vi "波形编辑.vi"(11 "db file":path=path "D:/Data/波形.sqlite3") -> (3 "波形图":waveform(dbl)(graph))   [LabVIEW 2020, in "功能选择.xctl"]
uses:
  <vilib>/drjdpowell/SQLite Library/SQL Statement/SQL Statement.lvclass/SQL Statement.ctl
  <vilib>/drjdpowell/SQLite Library/SQL Connection/Open (path).vi
  <vilib>/drjdpowell/SQLite Library/SQL Statement/Bind Text.vi
  <vilib>/drjdpowell/SQLite Library/SQL Statement/First Step.vi
  <vilib>/drjdpowell/SQLite Library/SQL Statement/Column DBL.vi
  <vilib>/drjdpowell/SQLite Library/SQL Statement/Finalize (Property).vi
  <vilib>/drjdpowell/SQLite Library/SQL Connection/Open (string).vi
  <vilib>/drjdpowell/SQLite Library/SQL Statement/Step.vi
  <vilib>/drjdpowell/SQLite Library/SQL Statement/Column Type.vi
  <vilib>/drjdpowell/SQLite Library/SQL Statement/Finalize.vi
  <vilib>/AdvancedString/Path To Command Line String.vi
  <vilib>/drjdpowell/SQLite Library/SQL Connection/Execute SQL (No results).vi
  <vilib>/Utility/file.llb/Write Delimited Spreadsheet (string).vi
  <vilib>/Utility/file.llb/Read Delimited Spreadsheet (string).vi
  <vilib>/drjdpowell/SQLite Library/SQL Statement/Error Message.vi
  <vilib>/drjdpowell/SQLite Library/SQL Statement/Column String.vi
  <vilib>/drjdpowell/SQLite Library/SQL Connection/Execute SQL (1D String).vi
  <vilib>/drjdpowell/SQLite Library/SQL Connection/Connection.lvclass
  <vilib>/drjdpowell/SQLite Library/SQL Statement/SQL Statement.lvclass
  <vilib>/drjdpowell/SQLite Library/SQLite.lvlib
panel:
  in  "limit I":dbl=0.01 min=1e-08 max=3.0 format="%#_6pA"
  in  "搜索":string
  out "保存列表":i32(listbox)
  in  "采样点（秒/个）":dbl=0.001 min=6.5e-05 max=1.0 step=1e-06 format="%#_6ps"
  in  "波形描述":string[][](table)=[["--------", "--end--", "--------", "--------"]]
  # "类型：\nL=线性  log=对数\nP=脉冲  S=阶跃"
  # "类型为对数时备注为渐近线线\n         脉冲时为占空比0-100\n         阶跃信号为突变位置0-100"
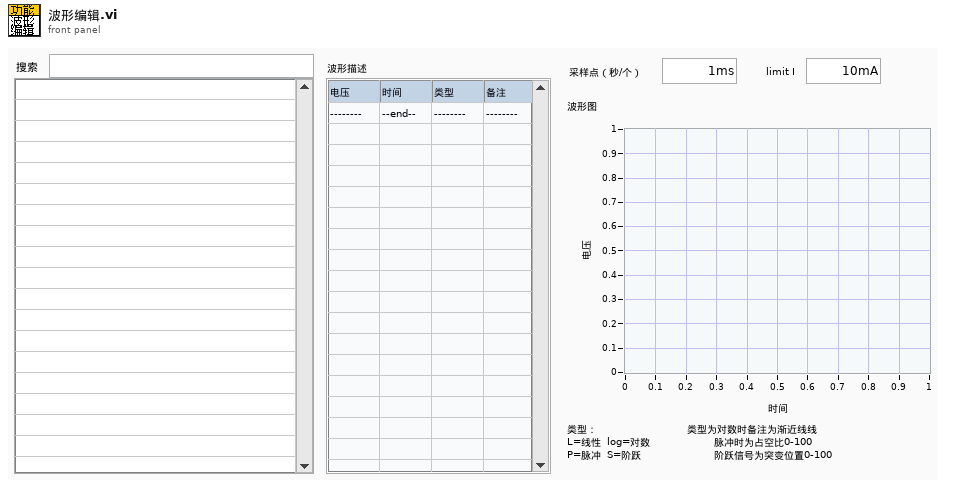
[diagram p1: front panel]
types:
  T1 = cluster{string, "采样点（秒/个）":dbl, "JSON string":string}
  T2 = typedef "LVPoint32TypeDef.ctl" = cluster{"Horizontal":i32, "Vertical":i32}
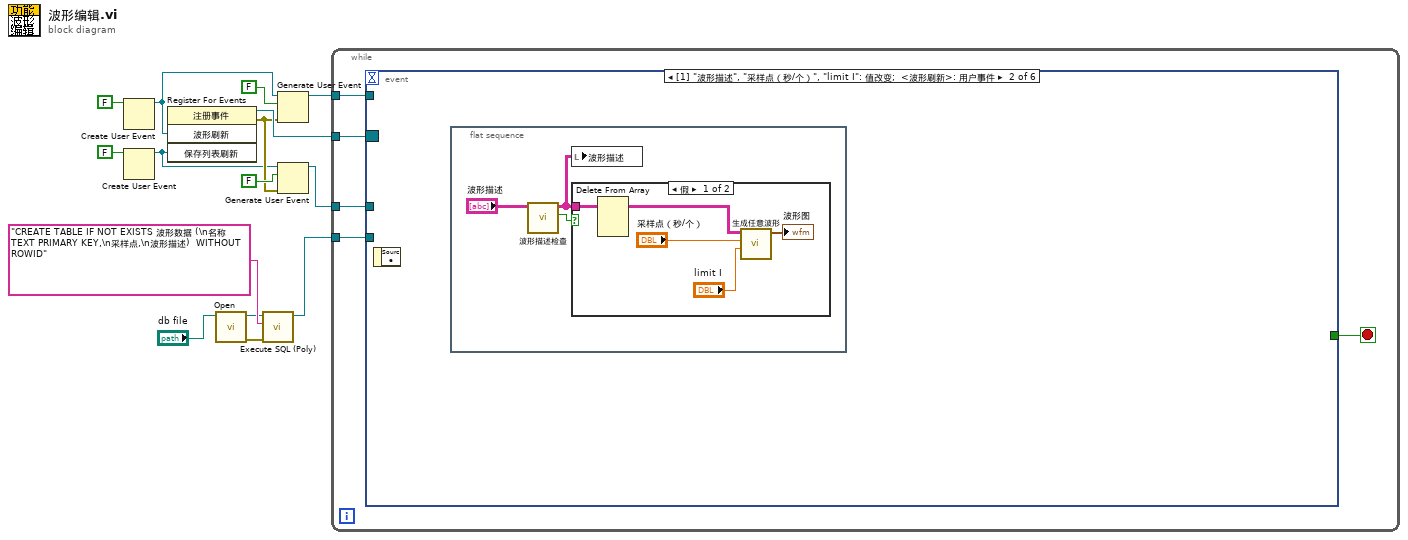
[diagram p0: block diagram]
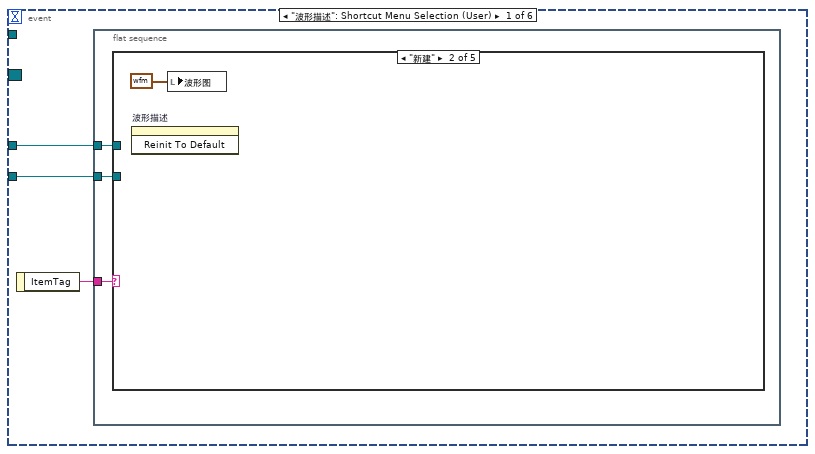
[diagram p2: hidden frame]
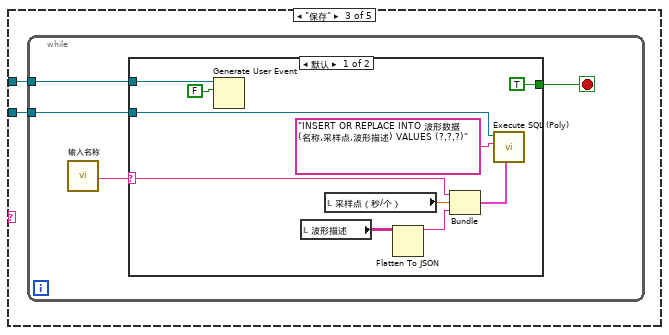
[diagram p4: hidden frame]
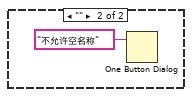
[diagram p5: hidden frame]
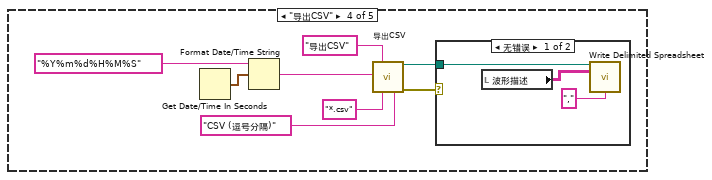
[diagram p6: hidden frame]
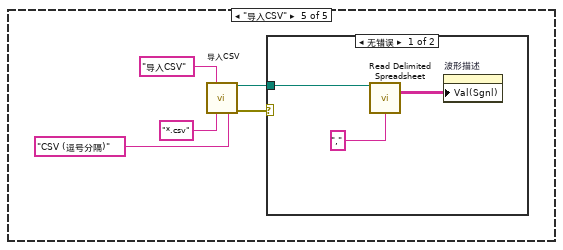
[diagram p8: hidden frame]
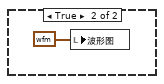
[diagram p10: hidden frame]
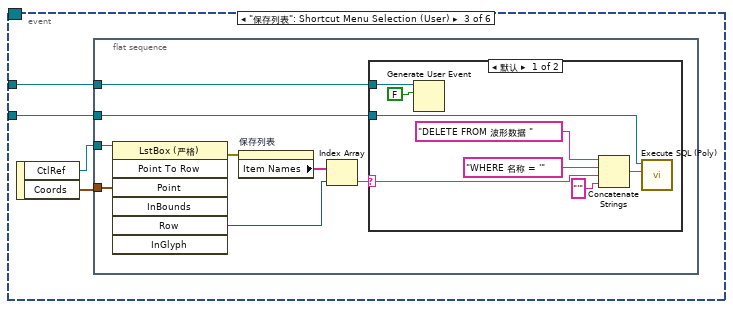
[diagram p11: hidden frame]
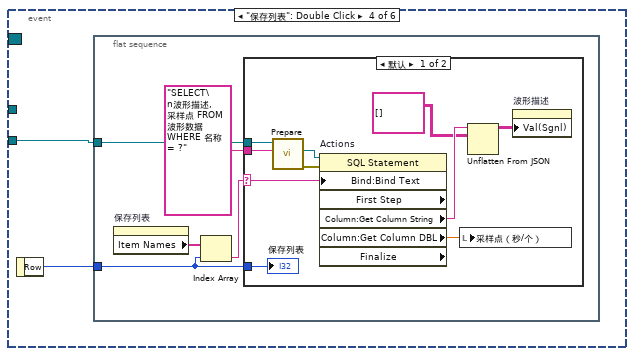
[diagram p13: hidden frame]
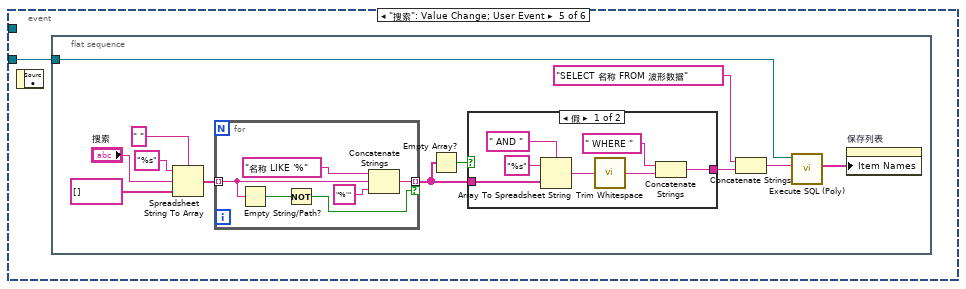
[diagram p15: hidden frame]
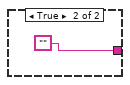
[diagram p16: hidden frame]
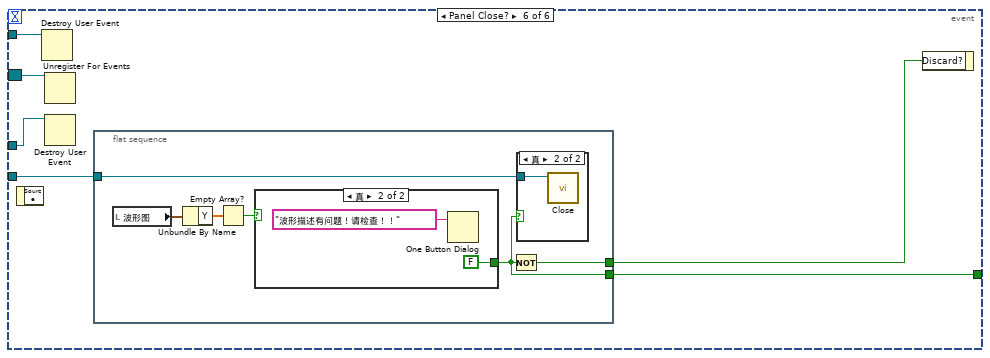
[diagram p17: hidden frame]
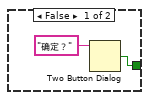
[diagram p19: hidden frame]
diagram:
  n1 = Create User Event(user event datatype=FALSE ("波形刷新")) -> (user event=w5:refnum<user-event>)  [unwired: 1 in, 1 out]
  n2 = Create User Event(user event datatype=FALSE ("保存列表刷新")) -> (user event=w3:refnum<user-event>)  [unwired: 1 in, 1 out]
  n3 = register-events(w5, w3) -> (reference out=w9:refnum<event-registration>, error out=w4:errorcluster)  [unwired: 2 in]
  n4 = call-poly <vilib>:"Open.vi"("db file"="db file") -> ("error out"=w11:errorcluster, "SQLite Connection"=w13:refnum<class "Connection.lvclass">)  [unwired: 9 in]
  n5 = call-poly <vilib>:"Execute SQL (Poly).vi"("error in (no error)"=w11, "SQL"="CREATE TABLE IF NOT EXISTS 波形数据 (\n名称 TEXT PRIMARY KEY,\n采样点,\n波形描述)  WITHOUT ROWID", "SQLite Connection in"=w13) -> ("SQLite Connection"=w12:refnum<class "Connection.lvclass">)  [unwired: 7 in, 1 out]
  n6 = Generate User Event(user event=w5, event data cluster=FALSE ("事件数据"), error in=w4) -> (user event out=w1:refnum<user-event>)  [unwired: 1 in, 1 out]
  n7 = Generate User Event(user event=w3, event data cluster=FALSE ("事件数据"), error in=w4) -> (user event out=w2:refnum<user-event>)  [unwired: 1 in, 1 out]
  n8 = while {
    tunnel: w12 -> [w19]
    tunnel: w9 -> [w18]
    tunnel: w2 -> [w17]
    tunnel: w1 -> [w16]
    stop <- w20 stop-if-true
    n9 = event shown="[1] \"波形描述\", \"采样点（秒/个）\", \"limit I\": 值改变;  <波形刷新>: 用户事件" {
      selector: w18 -> [_ _ _ _ _ w139]
      dyn-events: _ -> [_ _ _ _ _ _]
      timeout: _ -> [_ _ _ _ _ _]
      tunnel: [_ _ _ _ _ w141] -> w20
      tunnel: w19 -> [w22 _ w74 w93 w110 w142]
      tunnel: w17 -> [w21 _ w73 _ _ w138]
      tunnel: w16 -> [_ _ _ _ _ w137]
      event "波形描述": Shortcut Menu Selection (User) {
        n10 = event-data() -> ("ItemTag"=w23:string)  [unwired: 1 in]
        n11 = flat-sequence {
          tunnel: w23 -> [w26]
          tunnel: w22 -> [w25]
          tunnel: w21 -> [w24]
          frame #0 {
            n12 = case shown="\"新建\"" w26 {
              tunnel: w25 -> [_ _ w29 _ _]
              tunnel: w24 -> [_ _ w28 _ _]
              frame Default {
              }
              frame "新建" {
                n13 = invoke on="波形描述" class="Tbl (严格)" method="Reinit To Default"() -> ()  [unwired: 3 in, 3 out]
                n14 = local write "波形图"(waveform(dbl) {"t0"=timestamp(0 s since 1904-01-01), "dt"=1.0, "Y"=[]} ("波形图")) -> ()
              }
              frame "保存" {
                n15 = while {
                  tunnel: w29 -> [w33]
                  tunnel: w28 -> [w30]
                  stop <- w31 stop-if-true
                  n16 = call "输入名称"() -> ("名称"=w32:string)  [unwired: 17 in, 2 out]
                  n17 = case shown="默认" w32 {
                    selector: w32 -> [w36 _]
                    tunnel: w33 -> [w38 _]
                    tunnel: [TRUE _] -> w31
                    tunnel: w30 -> [w35 _]
                    frame Default {
                      n18 = Generate User Event(user event=w35, event data cluster=FALSE ("事件数据")) -> ()  [unwired: 2 in, 2 out]
                      n19 = local read "波形描述"() -> (w40:string[][])
                      n20 = local read "采样点（秒/个）"() -> (w42:dbl)
                      n21 = Flatten To JSON(anything=w40) -> (JSON string=w41:string)  [unwired: 2 in, 1 out]
                      n22 = Bundle(w36, "采样点（秒/个）"=w42, "JSON string"=w41) -> (w43:T1)  [unwired: 1 in]
                      n23 = call-poly <vilib>:"Execute SQL (Poly).vi"("Parameter(s)"=w43, "SQL"="INSERT OR REPLACE INTO 波形数据 (名称,采样点,波形描述) VALUES (?,?,?)", "SQLite Connection in"=w38) -> ()  [unwired: 7 in, 2 out]
                    }
                    frame "" {
                      n24 = One Button Dialog(message="不允许空名称" ("消息")) -> ()  [unwired: 1 in, 1 out]
                    }
                  }
                }
              }
              frame "导出CSV" {
                n25 = Get Date/Time In Seconds() -> (seconds since 1Jan1904=w49:timestamp)
                n26 = Format Date/Time String(time format string (%c)="%Y%m%d%H%M%S" ("时间格式字符串(%c)"), seconds (now)=w49) -> (date/time string=w48:string)  [unwired: 1 in]
                n27 = call "导出CSV"("prompt"="导出CSV", "default name"=w48, "pattern (all files)"="*.csv" ("pattern label"), "pattern label"="CSV (逗号分隔)" ("pattern (all files)")) -> ("selected path"=w52:path, "error out"=w46:errorcluster)  [unwired: 8 in, 2 out]
                n28 = case shown="无错误" w46 {
                  tunnel: w52 -> [w55 _]
                  frame No Error {
                    n29 = local read "波形描述"() -> (w54:string[][])
                    n30 = call-poly <vilib>:"Write Delimited Spreadsheet.vi"("file path (dialog if empty)"=w55, "2D data"=w54, "delimiter (\\t)"="," ("delimiter (\\t)")) -> ()  [unwired: 11 in, 2 out]
                  }
                  frame Error {
                  }
                }
              }
              frame "导入CSV" {
                n31 = call "导入CSV"("prompt"="导入CSV", "pattern (all files)"="*.csv" ("pattern label"), "pattern label"="CSV (逗号分隔)" ("pattern (all files)")) -> ("selected path"=w60:path, "error out"=w59:errorcluster)  [unwired: 9 in, 2 out]
                n32 = case shown="无错误" w59 {
                  tunnel: w60 -> [w63 _]
                  frame No Error {
                    n33 = call-poly <vilib>:"Read Delimited Spreadsheet.vi"("file path (dialog if empty)"=w63, "delimiter (\\t)"="," ("delimiter (\\t)")) -> ("all rows"=w61:string[][])  [unwired: 8 in, 5 out]
                    n34 = property on="波形描述" class="Tbl (严格)"("Val(Sgnl)"=w61) -> ()  [unwired: 2 in, 2 out]
                  }
                  frame Error {
                  }
                }
              }
            }
          }
        }
      }
      event "波形描述", "采样点（秒/个）", "limit I": Value Change; User Event {
        n35 = event-data() -> ()  [unwired: 1 in, 1 out]
        n36 = flat-sequence {
          frame #0 {
            n37 = call "波形描述检查.vi"("波形描述"="波形描述") -> ("正确"=w66:bool, "波形描述输出"=w64:string[][])  [unwired: 9 in]
            n38 = local write "波形描述"(w64) -> ()
            n39 = case shown="假" w66 {
              tunnel: w64 -> [w67 _]
              frame False {
                n40 = Delete From Array(array=w67) -> (array with subset deleted=w68:string[][])  [unwired: 3 in, 1 out]
                n41 = call "生成任意波形.vi"("限流"="limit I", "采样点"="采样点（秒/个）", "波形描述"=w68) -> ("波形图"=→"波形图":waveform(dbl))  [unwired: 8 in]
              }
              frame True {
                n42 = local write "波形图"(waveform(dbl) {"t0"=timestamp(0 s since 1904-01-01), "dt"=1.0, "Y"=[]} ("Waveform")) -> ()
              }
            }
          }
        }
      }
      event "保存列表": Shortcut Menu Selection (User) {
        n43 = event-data() -> ("CtlRef"=w76:refnum<vi>, "Coords"=w75:T2)  [unwired: 1 in]
        n44 = flat-sequence {
          tunnel: w76 -> [w84]
          tunnel: w75 -> [w83]
          tunnel: w74 -> [w79]
          tunnel: w73 -> [w77]
          frame #0 {
            n45 = invoke class="LstBox (严格)" method="Point To Row"(reference=w84, "Point"=w83) -> (error out=w78:errorcluster, "Row"=w81:i32)  [unwired: 5 in, 5 out]
            n46 = property on="保存列表" class="LstBox (严格)"(error in=w78) -> ("Item Names"=w82:string[])  [unwired: 1 in, 2 out]
            n47 = Index Array(array=w82, index=w81) -> (element=w80:string)
            n48 = case shown="默认" w80 {
              selector: w80 -> [w90 _]
              tunnel: w79 -> [w89 _]
              tunnel: w77 -> [w86 _]
              frame Default {
                n49 = Generate User Event(user event=w86, event data cluster=FALSE ("事件数据")) -> ()  [unwired: 2 in, 2 out]
                n50 = Concatenate Strings("DELETE FROM 波形数据 " ("字符串"), "WHERE 名称 = '" ("condition"), w90, "'" ("字符串")) -> (w87:string)
                n51 = call-poly <vilib>:"Execute SQL (Poly).vi"("SQL"=w87, "SQLite Connection in"=w89) -> ()  [unwired: 8 in, 2 out]
              }
              frame "" {
              }
            }
          }
        }
      }
      event "保存列表": Double Click {
        n52 = event-data() -> ("Row"=w94:i32)  [unwired: 1 in]
        n53 = flat-sequence {
          tunnel: w94 -> [w99]
          tunnel: w93 -> [w96]
          frame #0 {
            n54 = property on="保存列表" class="LstBox (严格)"() -> ("Item Names"=w98:string[])  [unwired: 2 in, 2 out]
            n55 = Index Array(array=w98, index=w99) -> (element=w97:string)
            n56 = case shown="默认" w97 {
              selector: w97 -> [w104 _]
              tunnel: w99 -> [w109 _]
              tunnel: w96 -> [w105 _]
              tunnel: "SELECT\n波形描述, 采样点 FROM 波形数据 WHERE 名称 = ?" ("SELECT  statement") -> [w102 _]
              frame Default {
                n57 = call <vilib>:"Prepare.vi"("SQL"=w102, "SQLite Connection in"=w105) -> ("error out"=w106:errorcluster, "SQL Statement"=w107:refnum<class "SQL Statement.lvclass">)  [unwired: 5 in, 3 out]
                n58 = property on="Actions" class="SQL Statement" props=["Bind:Bind Text", "First Step", "Column:Get Column String", "Column:Get Column DBL", "Finalize"](reference=w107, error in=w106, "Bind:Bind Text"=w104) -> ("Column:Get Column String"=w103:string, "Column:Get Column DBL"=w101:dbl)  [unwired: 4 out]
                n59 = local write "采样点（秒/个）"(w101) -> ()
                n60 = Unflatten From JSON(JSON string=w103, type and defaults=string[][] []) -> (value=w108:string[][])  [unwired: 5 in, 1 out]
                n61 = property on="波形描述" class="Tbl (严格)"("Val(Sgnl)"=w108) -> ()  [unwired: 2 in, 2 out]
                "保存列表" <- w109
              }
              frame "" {
              }
            }
          }
        }
      }
      event "搜索": Value Change; User Event {
        n62 = event-data() -> ()  [unwired: 1 in, 1 out]
        n63 = flat-sequence {
          tunnel: w110 -> [w111]
          frame #0 {
            n64 = Spreadsheet String To Array(delimiter (Tab)=" " ("分隔符(Tab)"), format string="%s" ("格式字符串"), spreadsheet string="搜索", array type (2D Dbl)=string[] []) -> (array=w118:string[])
            n65 = for {
              tunnel: w118 -> [w133] mode=indexing
              tunnel: [w134] -> w117 mode=indexing if=w131
              n66 = Empty String/Path?(string/path=w133) -> (empty?=w132:bool)
              n67 = Not(x=w132) -> (.not. x?=w131:bool)
              n68 = Concatenate Strings("名称 LIKE '%" ("字符串"), w133, "%'" ("condition")) -> (w134:string)
            }
            n69 = Empty Array?(array=w117) -> (empty?=w116:bool)
            n70 = case shown="假" w116 {
              tunnel: [w125 ""] -> w112
              tunnel: w117 -> [w123 _]
              frame False {
                n71 = Array To Spreadsheet String(delimiter (Tab)=" AND " ("分隔符(Tab)"), array=w123, 3:"%s" ("格式字符串")) -> (spreadsheet string=w127:string)
                n72 = call <vilib>:"Trim Whitespace.vi"("string"=w127) -> ("trimmed string"=w126:string)  [unwired: 1 in]
                n73 = Concatenate Strings(" WHERE ", w126) -> (w125:string)
              }
              frame True {
              }
            }
            n74 = Concatenate Strings("SELECT 名称 FROM 波形数据" ("SQL"), w112) -> (w113:string)
            n75 = call-poly <vilib>:"Execute SQL (Poly).vi"("SQL"=w113, "SQLite Connection in"=w111) -> ("Result Set"=w114:string[])  [unwired: 6 in, 3 out]
            n76 = property on="保存列表" class="LstBox (严格)"("Item Names"=w114) -> ()  [unwired: 2 in, 2 out]
          }
        }
      }
      event Panel Close? {
        n77 = event-data() -> ()  [unwired: 1 in, 1 out]
        n78 = Destroy User Event(user event=w137) -> ()  [unwired: 1 in, 1 out]
        n79 = Unregister For Events(event registration refnum=w139) -> ()  [unwired: 1 in, 1 out]
        n80 = Destroy User Event(user event=w138) -> ()  [unwired: 1 in, 1 out]
        n81 = flat-sequence {
          tunnel: w142 -> [w145]
          tunnel: [w144] -> w141
          tunnel: [w143] -> w140
          frame #0 {
            n82 = local read "波形图"() -> (w148:waveform(dbl))
            n83 = Unbundle By Name(w148) -> ("Y"=w147:dbl[])
            n84 = Empty Array?(array=w147) -> (empty?=w146:bool)
            n85 = case shown="真" w146 {
              tunnel: [w150 FALSE ("T button?")] -> w144
              frame False {
                n86 = Two Button Dialog(message="确定？" ("消息")) -> (T button?=w150:bool)  [unwired: 2 in]
              }
              frame True {
                n87 = One Button Dialog(message="波形描述有问题！请检查！！" ("消息")) -> ()  [unwired: 1 in, 1 out]
              }
            }
            n88 = Not(x=w144) -> (.not. x?=w143:bool)
            n89 = case shown="真" w144 {
              tunnel: w145 -> [_ w149]
              frame False {
              }
              frame True {
                n90 = call-dynamic "Close.vi"("SQLite Connection in"=w149) -> ()  [unwired: 10 in, 1 out]
              }
            }
          }
        }
        n91 = event-data("Discard?"=w140) -> ()  [unwired: 1 in, 1 out]
      }
    }
  }
